vi "Synced Example.vi"() -> ()   [LabVIEW 2020, in "2D Array Example.lvlib"]
uses:
  2D Array Example.lvlib
  OOPanel/2DArrayManager/2DArrayManager.lvclass
  2DArrayPanel/2DArrayPanel.lvclass
  OOPanel/Direction.ctl
  OOPanel/OOPanel.lvlib
  ExBlank/ExBlank.lvclass
panel:
  out "error out":errorcluster
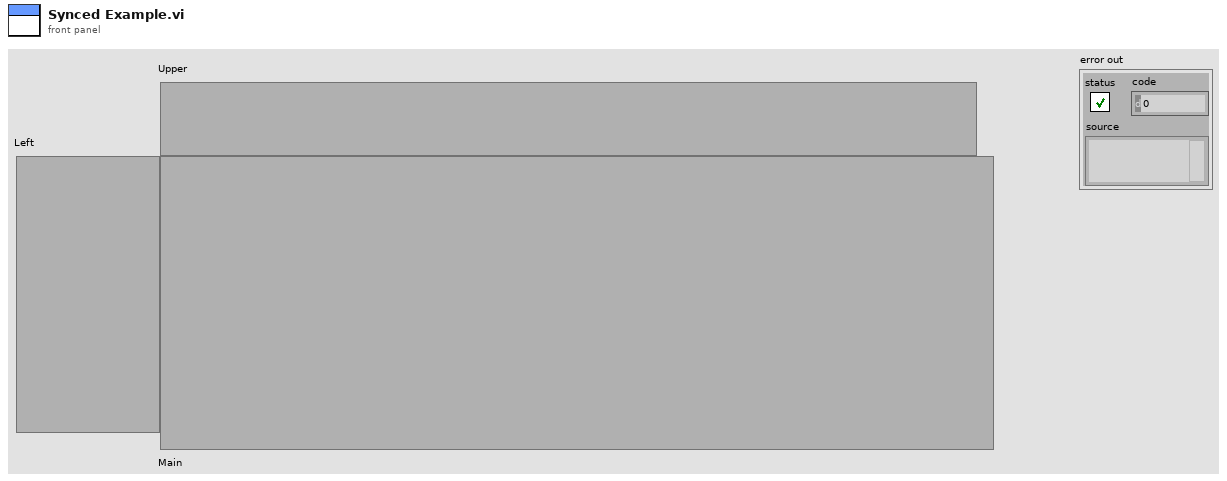
[diagram p1: front panel]
types:
  T1 = typedef "OOPanel.lvlib/Direction.ctl" = enum16{"Vertical", "Horizontal", "Both"}
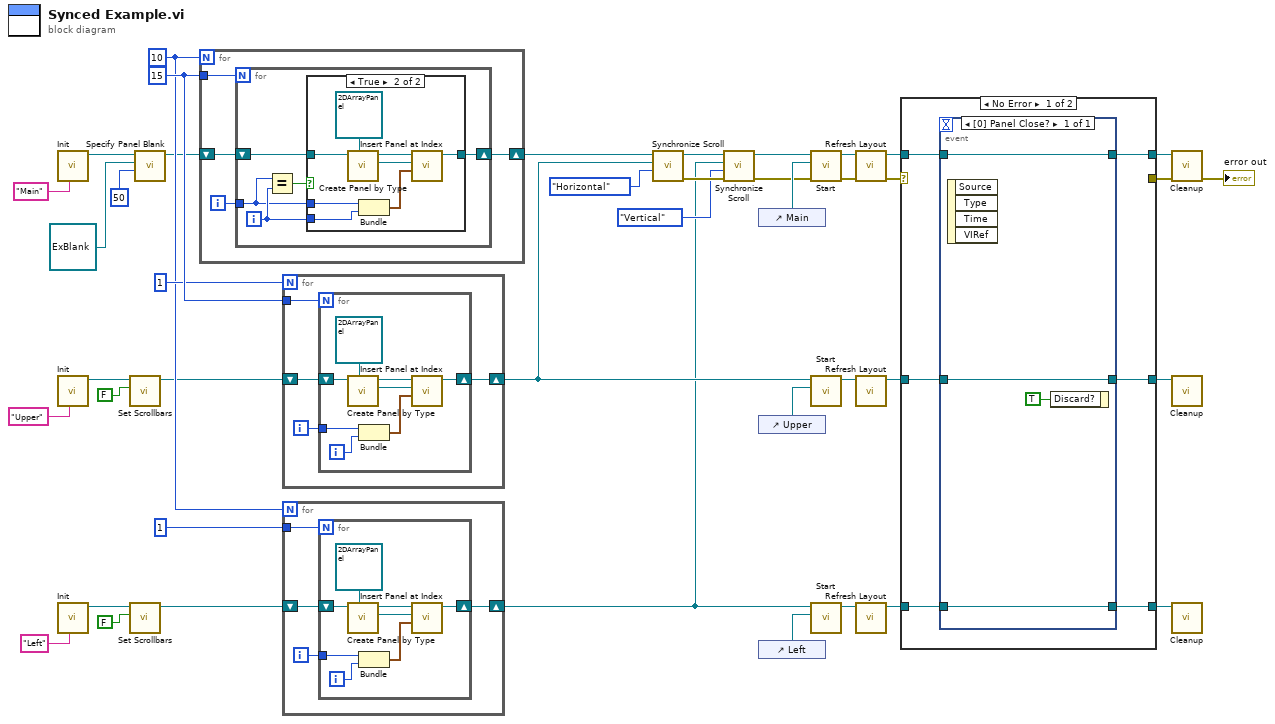
[diagram p0: block diagram]
diagram:
  w34 = 15
  w31 = 10
  n1 = call "Init.vi"("Name (Caller VI)"="Main") -> ("2DArrayManager out"=w37:refnum<class "2DArrayManager.lvclass">)  [unwired: 9 in, 1 out]
  n2 = call "Init.vi"("Name (Caller VI)"="Upper") -> ("2DArrayManager out"=w36:refnum<class "2DArrayManager.lvclass">)  [unwired: 9 in, 1 out]
  n3 = call "Init.vi"("Name (Caller VI)"="Left") -> ("2DArrayManager out"=w35:refnum<class "2DArrayManager.lvclass">)  [unwired: 9 in, 1 out]
  n4 = call "Set Scrollbars.vi"("Scrollbars"=FALSE, "2DArrayManager in"=w36) -> ("2DArrayManager out"=w10:refnum<class "2DArrayManager.lvclass">)  [unwired: 8 in, 1 out]
  n5 = call "Set Scrollbars.vi"("Scrollbars"=FALSE, "2DArrayManager in"=w35) -> ("2DArrayManager out"=w9:refnum<class "2DArrayManager.lvclass">)  [unwired: 8 in, 1 out]
  n6 = call "Specify Panel Blank.vi"("Initial Blank Count (0)"=50, "Blank VI"=refnum<class "ExBlank.lvclass"> refnum ("2D Array Example.lvlib:ExBlank.lvclass"), "2DArrayManager in"=w37) -> ("2DArrayManager out"=w6:refnum<class "2DArrayManager.lvclass">)  [unwired: 7 in, 1 out]
  n7 = for {
    N: w31 -> [_]
    tunnel: w34 -> [w46]
    shift-right: [w44] -> w30
    shift-left: w6 -> [w45]
    i -> [w43]
    n8 = for {
      N: w46 -> [_]
      shift-right: [w50] -> w44
      shift-left: w45 -> [w51]
      tunnel: w43 -> [w48]
      i -> [w49]
      n9 = Equal?(x=w48, y=w49) -> (x = y?=w47:bool)
      n10 = case shown="True" w47 {
        tunnel: w51 -> [w52 w60]
        tunnel: [w52 w55] -> w50
        tunnel: w49 -> [_ w54]
        tunnel: w48 -> [_ w53]
        frame False {
        }
        frame True {
          n11 = call "Create Panel by Type.vi"("Panel Type"=refnum<class "2DArrayPanel.lvclass"> refnum ("2D Array Example.lvlib:2DArrayPanel.lvclass"), "2DArrayManager in"=w60) -> ("Panel"=w57:refnum<class "2DArrayPanel.lvclass">, "2DArrayManager out"=w58:refnum<class "2DArrayManager.lvclass">)  [unwired: 7 in, 1 out]
          n12 = Bundle(w53, w54) -> (w56:cluster{i32, i32})  [unwired: 1 in]
          n13 = call "Insert Panel at Index.vi"("2D Index"=w56, "ArrayPanel"=w57, "2DArrayManager in"=w58) -> ("2DArrayManager out"=w55:refnum<class "2DArrayManager.lvclass">)  [unwired: 5 in, 3 out]
        }
      }
    }
  }
  n14 = for {
    N: 1 -> [_]
    tunnel: w34 -> [w64]
    shift-right: [w62] -> w25
    shift-left: w10 -> [w63]
    i -> [w61]
    n15 = for {
      N: w64 -> [_]
      shift-right: [w65] -> w62
      shift-left: w63 -> [w70]
      tunnel: w61 -> [w72]
      i -> [w71]
      n16 = call "Create Panel by Type.vi"("Panel Type"=refnum<class "2DArrayPanel.lvclass"> refnum ("2D Array Example.lvlib:2DArrayPanel.lvclass"), "2DArrayManager in"=w70) -> ("Panel"=w67:refnum<class "2DArrayPanel.lvclass">, "2DArrayManager out"=w68:refnum<class "2DArrayManager.lvclass">)  [unwired: 7 in, 1 out]
      n17 = Bundle(w72, w71) -> (w66:cluster{i32, i32})  [unwired: 1 in]
      n18 = call "Insert Panel at Index.vi"("2D Index"=w66, "ArrayPanel"=w67, "2DArrayManager in"=w68) -> ("2DArrayManager out"=w65:refnum<class "2DArrayManager.lvclass">)  [unwired: 5 in, 3 out]
    }
  }
  n19 = for {
    N: w31 -> [_]
    tunnel: 1 -> [w76]
    shift-right: [w74] -> w2
    shift-left: w9 -> [w75]
    i -> [w73]
    n20 = for {
      N: w76 -> [_]
      shift-right: [w77] -> w74
      shift-left: w75 -> [w82]
      tunnel: w73 -> [w84]
      i -> [w83]
      n21 = call "Create Panel by Type.vi"("Panel Type"=refnum<class "2DArrayPanel.lvclass"> refnum ("2D Array Example.lvlib:2DArrayPanel.lvclass"), "2DArrayManager in"=w82) -> ("Panel"=w79:refnum<class "2DArrayPanel.lvclass">, "2DArrayManager out"=w80:refnum<class "2DArrayManager.lvclass">)  [unwired: 7 in, 1 out]
      n22 = Bundle(w84, w83) -> (w78:cluster{i32, i32})  [unwired: 1 in]
      n23 = call "Insert Panel at Index.vi"("2D Index"=w78, "ArrayPanel"=w79, "2DArrayManager in"=w80) -> ("2DArrayManager out"=w77:refnum<class "2DArrayManager.lvclass">)  [unwired: 5 in, 3 out]
    }
  }
  n24 = call "Synchronize Scroll.vi"("Direction"=Direction."Horizontal", "Other 2D Array"=w25, "2DArrayManager in"=w30) -> ("error out"=w41:errorcluster, "2DArrayManager out"=w28:refnum<class "2DArrayManager.lvclass">)  [unwired: 7 in]
  n25 = call "Synchronize Scroll.vi"("error in (no error)"=w41, "Direction"=Direction."Vertical", "Other 2D Array"=w2, "2DArrayManager in"=w28) -> ("error out"=w19:errorcluster, "2DArrayManager out"=w4:refnum<class "2DArrayManager.lvclass">)  [unwired: 6 in]
  n26 = control-ref of="Main"() -> (w26:refnum<vi>)
  n27 = control-ref of="Upper"() -> (w24:refnum<vi>)
  n28 = control-ref of="Left"() -> (w23:refnum<vi>)
  n29 = call "Start.vi"("error in (no error)"=w19, "Container"=w26, "2DArrayManager in"=w4) -> ("error out"=w3:errorcluster, "2DArrayManager out"=w20:refnum<class "2DArrayManager.lvclass">)  [unwired: 7 in]
  n30 = call "Start.vi"("Container"=w24, "2DArrayManager in"=w25) -> ("2DArrayManager out"=w21:refnum<class "2DArrayManager.lvclass">)  [unwired: 8 in, 1 out]
  n31 = call "Start.vi"("Container"=w23, "2DArrayManager in"=w2) -> ("2DArrayManager out"=w22:refnum<class "2DArrayManager.lvclass">)  [unwired: 8 in, 1 out]
  n32 = call "Refresh Layout.vi"("error in (no error)"=w3, "2DArrayManager in"=w20) -> ("error out"=w18:errorcluster, "2DArrayManager out"=w17:refnum<class "2DArrayManager.lvclass">)  [unwired: 8 in]
  n33 = call "Refresh Layout.vi"("2DArrayManager in"=w21) -> ("2DArrayManager out"=w16:refnum<class "2DArrayManager.lvclass">)  [unwired: 9 in, 1 out]
  n34 = call "Refresh Layout.vi"("2DArrayManager in"=w22) -> ("2DArrayManager out"=w15:refnum<class "2DArrayManager.lvclass">)  [unwired: 9 in, 1 out]
  n35 = case shown="No Error" w18 {
    selector: w18 -> [_ w95]
    tunnel: w17 -> [w85 w98]
    tunnel: w16 -> [w87 w97]
    tunnel: w15 -> [w89 w96]
    tunnel: [w90 w96] -> w13
    tunnel: [w88 w97] -> w12
    tunnel: [w86 w98] -> w14
    tunnel: [_ w95] -> w11
    frame No Error {
      n36 = event shown="[0] Panel Close?" {
        selector: _ -> [_]
        dyn-events: _ -> [_]
        timeout: _ -> [_]
        tunnel: [w94] -> w90
        tunnel: w89 -> [w94]
        tunnel: [w93] -> w88
        tunnel: w87 -> [w93]
        tunnel: [w92] -> w86
        tunnel: w85 -> [w92]
        event Panel Close? {
          n37 = event-data() -> ()  [unwired: 1 in, 4 out]
          n38 = event-data("Discard?"=TRUE) -> ()  [unwired: 1 in, 1 out]
        }
      }
    }
    frame Error {
    }
  }
  n39 = call "Cleanup.vi"("error in (no error)"=w11, "2DArrayManager in"=w14) -> ("error out"=→"error out":errorcluster)  [unwired: 9 in]
  n40 = call "Cleanup.vi"("2DArrayManager in"=w12) -> ()  [unwired: 10 in, 1 out]
  n41 = call "Cleanup.vi"("2DArrayManager in"=w13) -> ()  [unwired: 10 in, 1 out]
